vi "to string.vi"(8 "error in":errorcluster, 11 "Shared Memory configuration in":refnum<class "Shared Memory configuration.lvclass">) -> (0 "error out":errorcluster, 1 "data":string, 2 "version":string, 3 "Shared Memory configuration out":refnum<class "Shared Memory configuration.lvclass">)   [LabVIEW 2014, in "Shared Memory configuration.lvclass"]
doc: "Provides an interface for saving a module configuration to a file or other serialized data source. It is recommended that all children of this class store data in two sets--data required for its own initialization, and any data required for parent initialization--and that each implementation uses the <b>Call Parent Method</b> primitive to serialize parent information."
uses:
  Shared Memory configuration.lvclass
  current version.vi
  <vilib>/NI/Tag Bus Module Framework/module configuration/TBM module configuration.lvclass
  <vilib>/NI/Configuration Framework/serializable configuration/NISE_CEF_serializable configuration.lvclass
  <vilib>/NI/Tag Bus Module Framework/channel/TBM channel.lvclass
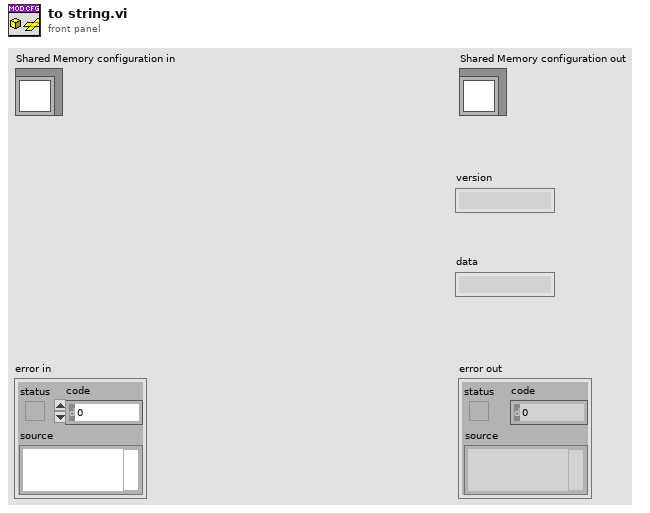
[diagram p1: front panel]
types:
  T1 = typedef "Shared Memory configuration.lvclass/Line.ctl" = cluster{"channel":refnum<class "TBM channel.lvclass">}
  T2 = typedef "Shared Memory configuration.lvclass/sync item.ctl" = cluster{"mechanism":T3, "name":string}
  T3 = typedef "Shared Memory configuration.lvclass/sync mechanism.ctl" = enum16{"Semaphore"}
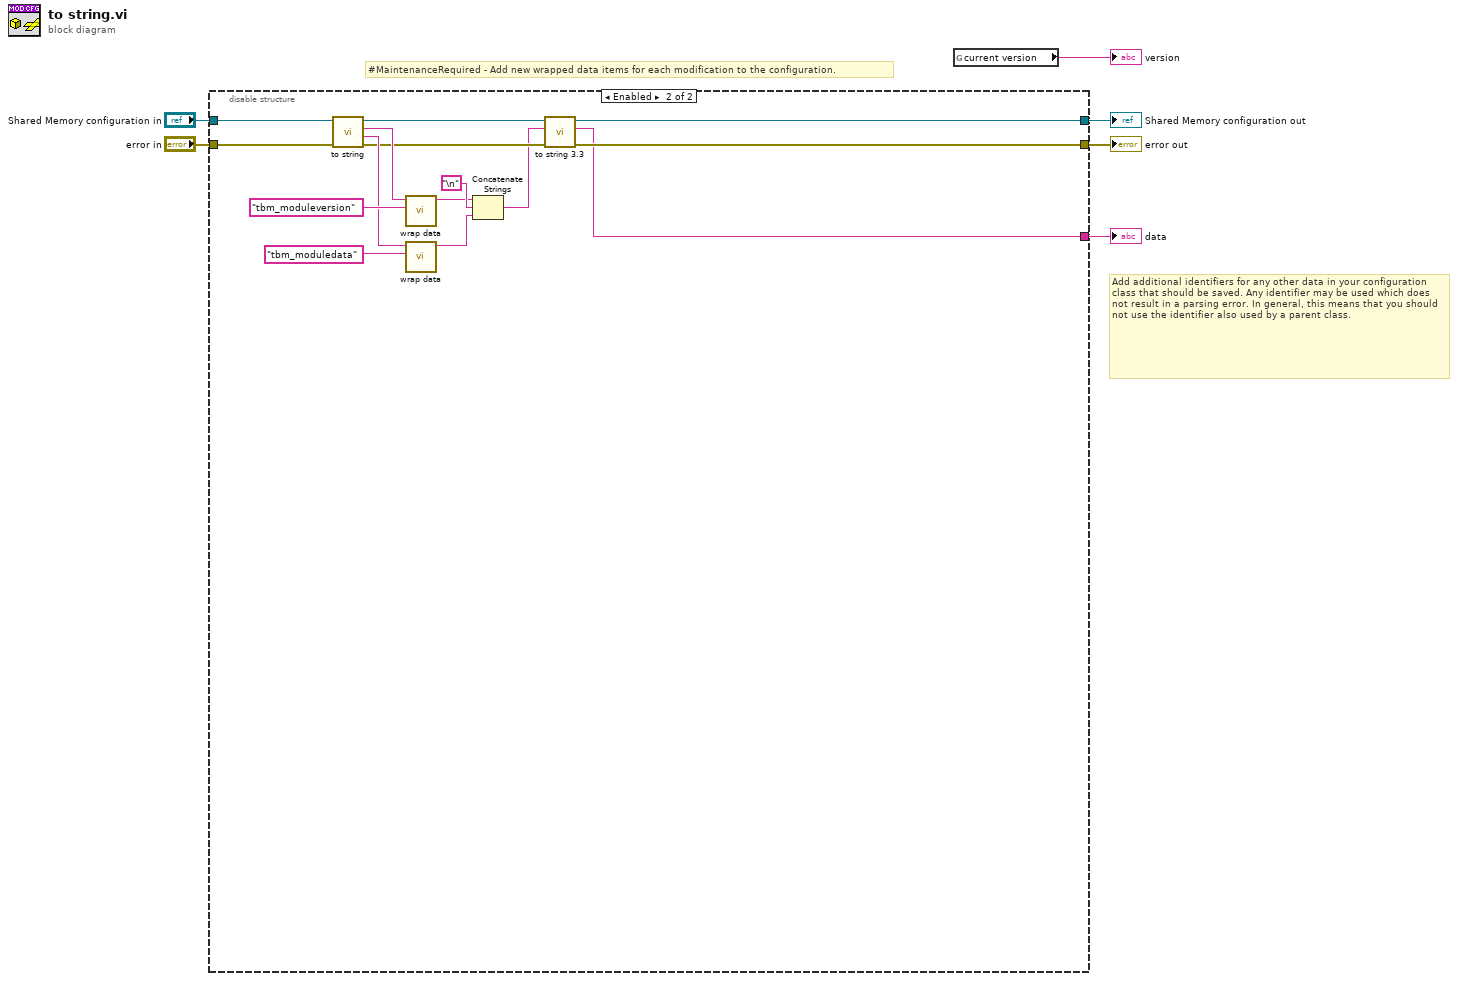
[diagram p0: block diagram]
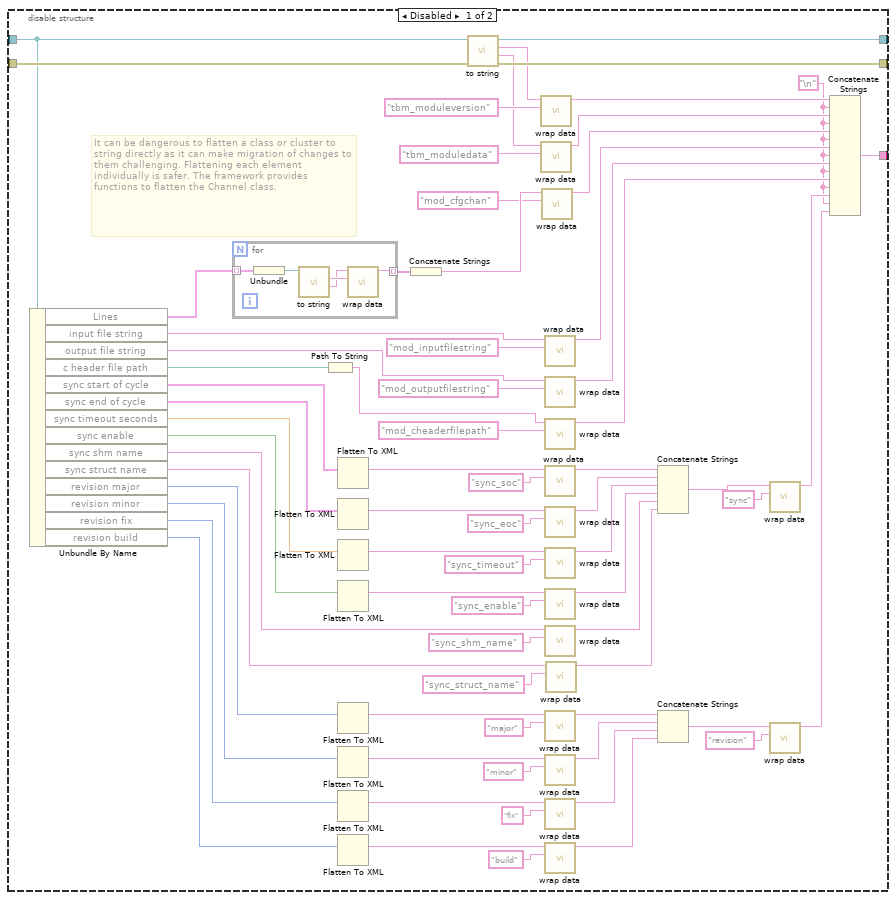
[diagram p2: hidden frame]
diagram:
  # "#MaintenanceRequired - Add new wrapped data items for each modification to the configuration."
  # "Add additional identifiers for any other data in your configuration class that should be saved. Any identifier may be used which does not result in a parsing error. In general, this means that you should not use the identifier also used by a parent class."
  n1 = disable-structure shown="Enabled" {
    disable-tunnel: "error in" -> [w77 w94]
    disable-tunnel: [w76 w86] -> w4
    disable-tunnel: [w75 w87] -> w3
    disable-tunnel: [w68 w83] -> w2
    disable-tunnel: "Shared Memory configuration in" -> [w67 w95]
    frame Disabled {
      w12 = "\n"
      # "It can be dangerous to flatten a class or cluster to string directly as it can make migration of changes to them challenging. Flattening each element individually is safer. The framework provides functions to flatten the Channel class."
      n2 = Unbundle By Name(w67) -> ("Lines"=w65:T1[], "input file string"=w58:string, "output file string"=w57:string, "c header file path"=w56:path, "sync start of cycle"=w42:T2[], "sync end of cycle"=w50:T2[], "sync timeout seconds"=w45:dbl, "sync enable"=w41:bool, "sync shm name"=w38:string, "sync struct name"=w8:string, "revision major"=w11:u16, "revision minor"=w29:u16, "revision fix"=w28:u16, "revision build"=w27:u16)
      n3 = for {
        tunnel: w65 -> [w82] mode=indexing
        tunnel: [w78] -> w64 mode=indexing
        n4 = Unbundle(w82) -> ("channel"=w81:refnum<class "TBM channel.lvclass">)
        n5 = call-dynamic "to string.vi"("channel in"=w81) -> ("channel data"=w79:string, "identifier"=w80:string)  [unwired: 7 in, 2 out]
        n6 = call <vilib>:"wrap data.vi"("identifier"=w80, "data to wrap"=w79) -> ("wrapped data"=w78:string)  [unwired: 9 in]
      }
      n7 = Path To String(path=w56) -> (string=w55:string)
      n8 = Flatten To XML(anything=w42) -> (xml string=w49:string)
      n9 = Flatten To XML(anything=w50) -> (xml string=w47:string)
      n10 = Flatten To XML(anything=w45) -> (xml string=w44:string)
      n11 = Flatten To XML(anything=w41) -> (xml string=w40:string)
      n12 = Flatten To XML(anything=w11) -> (xml string=w33:string)
      n13 = Flatten To XML(anything=w29) -> (xml string=w30:string)
      n14 = Flatten To XML(anything=w28) -> (xml string=w31:string)
      n15 = Flatten To XML(anything=w27) -> (xml string=w32:string)
      n16 = Concatenate Strings(w64) -> (w63:string)
      n17 = call-parent "to string.vi"("error in"=w77, "module configuration in"=w67) -> ("error out"=w75:errorcluster, "data"=w69:string, "version"=w70:string, "module configuration out"=w76:refnum<class "Shared Memory configuration.lvclass">)  [unwired: 6 in]
      n18 = call <vilib>:"wrap data.vi"("identifier"="tbm_moduleversion" ("additional identifier"), "data to wrap"=w70) -> ("wrapped data"=w72:string)  [unwired: 9 in]
      n19 = call <vilib>:"wrap data.vi"("identifier"="tbm_moduledata" ("additional identifier"), "data to wrap"=w69) -> ("wrapped data"=w71:string)  [unwired: 9 in]
      n20 = call <vilib>:"wrap data.vi"("identifier"="mod_cfgchan", "data to wrap"=w63) -> ("wrapped data"=w66:string)  [unwired: 9 in]
      n21 = call <vilib>:"wrap data.vi"("identifier"="mod_inputfilestring", "data to wrap"=w58) -> ("wrapped data"=w54:string)  [unwired: 9 in]
      n22 = call <vilib>:"wrap data.vi"("identifier"="mod_outputfilestring", "data to wrap"=w57) -> ("wrapped data"=w53:string)  [unwired: 9 in]
      n23 = call <vilib>:"wrap data.vi"("identifier"="mod_cheaderfilepath", "data to wrap"=w55) -> ("wrapped data"=w52:string)  [unwired: 9 in]
      n24 = call <vilib>:"wrap data.vi"("identifier"="sync_soc", "data to wrap"=w49) -> ("wrapped data"=w25:string)  [unwired: 9 in]
      n25 = call <vilib>:"wrap data.vi"("identifier"="sync_eoc", "data to wrap"=w47) -> ("wrapped data"=w24:string)  [unwired: 9 in]
      n26 = call <vilib>:"wrap data.vi"("identifier"="sync_timeout", "data to wrap"=w44) -> ("wrapped data"=w23:string)  [unwired: 9 in]
      n27 = call <vilib>:"wrap data.vi"("identifier"="sync_enable", "data to wrap"=w40) -> ("wrapped data"=w22:string)  [unwired: 9 in]
      n28 = call <vilib>:"wrap data.vi"("identifier"="sync_shm_name", "data to wrap"=w38) -> ("wrapped data"=w21:string)  [unwired: 9 in]
      n29 = call <vilib>:"wrap data.vi"("identifier"="major", "data to wrap"=w33) -> ("wrapped data"=w19:string)  [unwired: 9 in]
      n30 = call <vilib>:"wrap data.vi"("identifier"="minor", "data to wrap"=w30) -> ("wrapped data"=w18:string)  [unwired: 9 in]
      n31 = call <vilib>:"wrap data.vi"("identifier"="fix", "data to wrap"=w31) -> ("wrapped data"=w17:string)  [unwired: 9 in]
      n32 = call <vilib>:"wrap data.vi"("identifier"="build", "data to wrap"=w32) -> ("wrapped data"=w16:string)  [unwired: 9 in]
      n33 = call <vilib>:"wrap data.vi"("identifier"="sync_struct_name", "data to wrap"=w8) -> ("wrapped data"=w7:string)  [unwired: 9 in]
      n34 = Concatenate Strings(w25, w24, w23, w22, w21, w7) -> (w20:string)
      n35 = Concatenate Strings(w19, w18, w17, w16) -> (w15:string)
      n36 = call <vilib>:"wrap data.vi"("identifier"="sync", "data to wrap"=w20) -> ("wrapped data"=w14:string)  [unwired: 9 in]
      n37 = call <vilib>:"wrap data.vi"("identifier"="revision", "data to wrap"=w15) -> ("wrapped data"=w13:string)  [unwired: 9 in]
      n38 = Concatenate Strings(w72, w12, w71, w12, w66, w12, w54, w12, w53, w12, w52, w12, w14, w12, w13) -> (w68:string)
    }
    frame Enabled {
      n39 = call-parent "to string.vi"("error in"=w94, "module configuration in"=w95) -> ("error out"=w88:errorcluster, "data"=w92:string, "version"=w93:string, "module configuration out"=w85:refnum<class "Shared Memory configuration.lvclass">)  [unwired: 6 in]
      n40 = call <vilib>:"wrap data.vi"("identifier"="tbm_moduleversion" ("additional identifier"), "data to wrap"=w93) -> ("wrapped data"=w89:string)  [unwired: 9 in]
      n41 = call <vilib>:"wrap data.vi"("identifier"="tbm_moduledata" ("additional identifier"), "data to wrap"=w92) -> ("wrapped data"=w91:string)  [unwired: 9 in]
      n42 = Concatenate Strings(w89, "\n", w91) -> (w84:string)
      n43 = call "to string 3.3.vi"("error in"=w88, "data in"=w84, "Shared Memory configuration in"=w85) -> ("error out"=w87:errorcluster, "data out"=w83:string, "Shared Memory configuration out"=w86:refnum<class "Shared Memory configuration.lvclass">)  [unwired: 6 in]
    }
  }
  "error out" <- w3
  "Shared Memory configuration out" <- w4
  "data" <- w2
  n44 = global read "current version.vi" "current version"() -> (→"version":string)
